vi "GOOP_LVClass_Item_OnPopUpMenu.vi"(11 "Object":u64) -> ()   [LabVIEW 2020]
uses:
  <resource>/Framework/Providers/API/mxLvMenuItem.ctl
  <resource>/Framework/Providers/Open_GDS/ClassProviders/Provider_EndevoGOOP300/EndevoProviderName.ctl
  <resource>/Framework/Providers/Open_GDS/ClassProviders/Provider_EndevoGOOP400/EndevoG4ProviderName.ctl
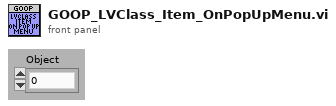
[diagram p1: front panel]
types:
  T1 = typedef "mxLvMenuItem.ctl" = cluster{"Menu Name":string, "Description":string, "Icon File Name":path, "Menu Tag":string, "Enabled":bool, "Checked":bool, "Separator":bool, "Batchable":bool, "Weight":i32, "Batch Mode (Ignored if Not Batchable)":enum32{"Show If All Items Support Command", "Show If Any Items Support Command"}, "Menu Location":enum32{"<None>", "Project", "Project / Build Specifications", "Tools", "Tools / Source Control", "Tools / Real-Time Module", "Help"}, "Exclude From Getting Started Window Menu":bool}
  T2 = typedef "EndevoG4ProviderName.ctl" = enum16{"EndevoGOOP400"}
  T3 = typedef "EndevoProviderName.ctl" = enum16{"EndevoGOOP300"}
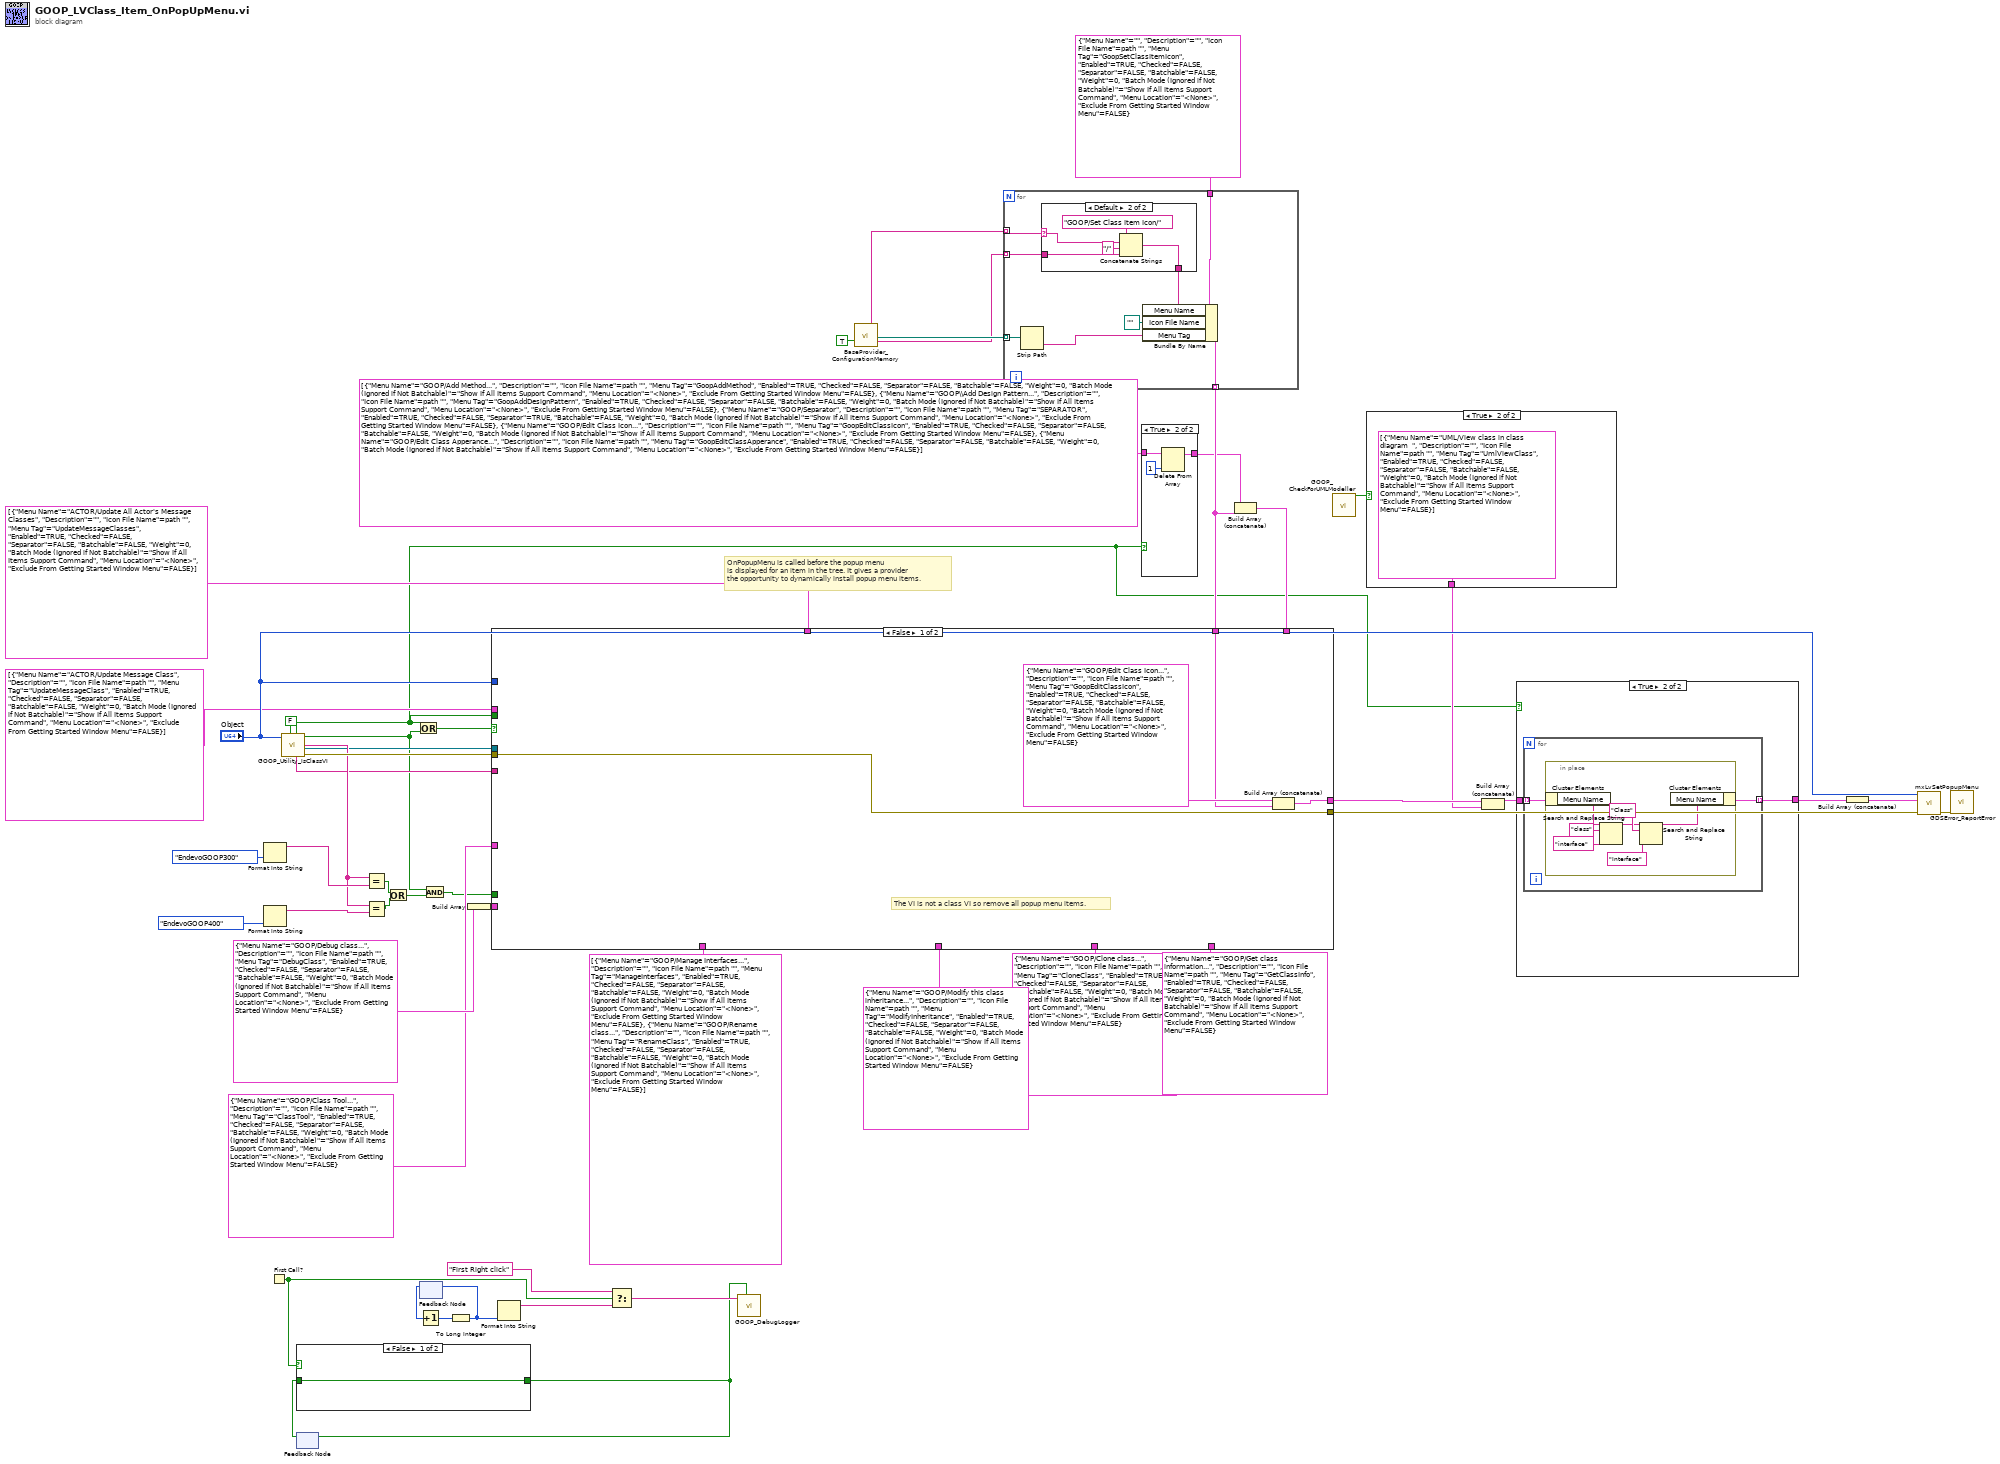
[diagram p0: block diagram]
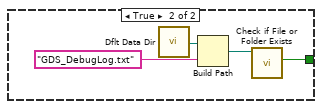
[diagram p5: hidden frame]
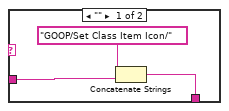
[diagram p6: hidden frame]
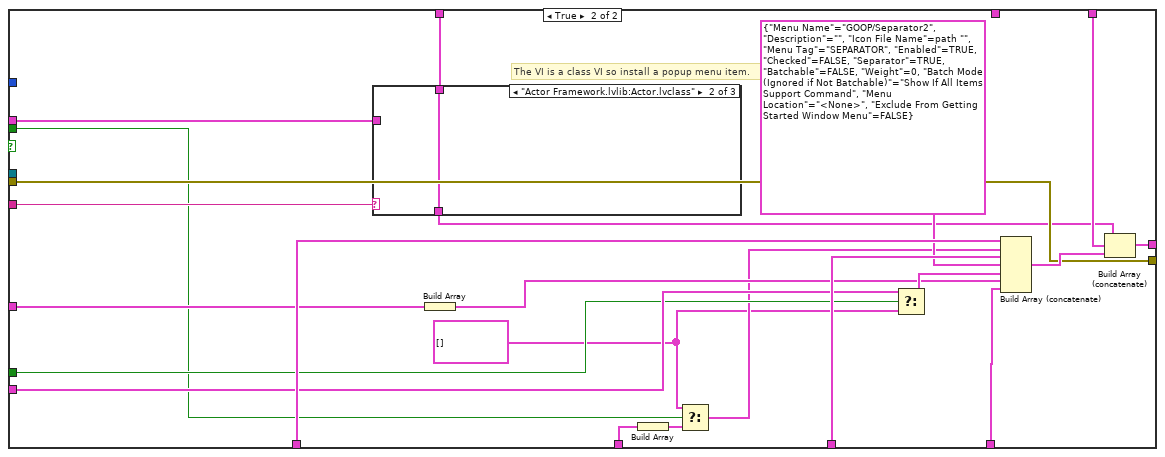
[diagram p7: hidden frame]
diagram:
  # "OnPopupMenu is called before the popup menu\nis displayed for an item in the tree. It gives a provider\nthe opportunity to dynamically install popup menu items."
  n1 = Format Into String(EndevoProviderName."EndevoGOOP300" ("ProviderName")) -> (resulting string=w34:string)  [unwired: 3 in, 1 out]
  n2 = Format Into String(EndevoG4ProviderName."EndevoGOOP400" ("ProviderName")) -> (resulting string=w31:string)  [unwired: 3 in, 1 out]
  n3 = First Call?() -> (First Call?: T/F=w20:bool)
  n4 = call <resource>:"GOOP_Utility_IsClassVI.vi"("KeepClassOpen(False)"=FALSE, "Object"="Object") -> ("error out"=w51:errorcluster, "ClassItem(If Found)"=w13:refnum<vi>, "ClassProvider"=w32:string, "Is Class VI?"=w8:bool, "RootClassQualified Class Name"=w18:string, "Is Interface?"=w3:bool)  [unwired: 4 in]
  n5 = feedback #1() -> (w21:bool)  [unwired: 1 in]
  n6 = case shown="False" w20 {
    tunnel: [w53 w54] -> w19
    tunnel: w21 -> [w53 _]
    frame False {
    }
    frame True {
      n7 = call <vilib>:"Dflt Data Dir.vi"() -> ("App:Default Data Directory"=w56:path)
      n8 = Build Path(base path=w56, name or relative path="GDS_DebugLog.txt") -> (appended path=w57:path)
      n9 = call <vilib>:"Check if File or Folder Exists.vi"("path"=w57) -> ("file or folder exists?"=w54:bool)  [unwired: 8 in, 2 out]
    }
  }
  n10 = feedback-in #1(w19) -> ()
  n11 = Equal?(x=w32, y=w34) -> (x = y?=w29:bool)
  n12 = Equal?(x=w32, y=w31) -> (x = y?=w30:bool)
  n13 = Or(x=w29, y=w30) -> (x .or. y?=w10:bool)
  n14 = Or(x=w3, y=w8) -> (x .or. y?=w11:bool)
  n15 = feedback #2() -> (w25:i32)  [unwired: 1 in]
  n16 = Increment(x=w25) -> (x+1=w24:i32)
  n17 = And(x=w8, y=w10) -> (x .and. y?=w9:bool)
  n18 = To Long Integer(number=w24) -> (32bit integer=w23:i32)
  n19 = feedback-in #2(w23) -> ()
  n20 = Build Array(T1 {"Menu Name"="GOOP/Debug class...", "Description"="", "Icon File Name"=path "", "Menu Tag"="DebugClass", "Enabled"=TRUE, "Checked"=FALSE, "Separator"=FALSE, "Batchable"=FALSE, "Weight"=0, "Batch Mode (Ignored if Not Batchable)"=enum."Show If All Items Support Command", "Menu Location"=enum."<None>", "Exclude From Getting Started Window Menu"=FALSE} ("Menu Item")) -> (w35:T1[])
  n21 = Format Into String(w23) -> (resulting string=w22:string)  [unwired: 3 in, 1 out]
  n22 = Select(t="First Right click" ("name or relative path"), s=w20, f=w22) -> (s? t:f=w27:string)
  n23 = call <resource>:"GOOP_DebugLogger.vi"("ActivateDebugging"=w19, "State"=w27) -> ()  [unwired: 7 in, 3 out]
  n24 = call <resource>:"BaseProvider_ConfigurationMemory.vi"("Filter_Icons"=TRUE) -> ("ClassItemIconGroup"=w28:string[], "ClassItemIconPaths"=w38:path[], "ClassItemIconNames"=w37:string[])  [unwired: 12 in, 4 out]
  n25 = for {
    tunnel: [w64] -> w40 mode=indexing
    tunnel: T1 {"Menu Name"="", "Description"="", "Icon File Name"=path "", "Menu Tag"="GoopSetClassItemIcon", "Enabled"=TRUE, "Checked"=FALSE, "Separator"=FALSE, "Batchable"=FALSE, "Weight"=0, "Batch Mode (Ignored if Not Batchable)"=enum."Show If All Items Support Command", "Menu Location"=enum."<None>", "Exclude From Getting Started Window Menu"=FALSE} ("Menu Item") -> [w65]
    tunnel: w38 -> [w61] mode=indexing
    tunnel: w37 -> [w59] mode=indexing
    tunnel: w28 -> [w58] mode=indexing
    n26 = Strip Path(path=w61) -> (name=w60:string)  [unwired: 1 out]
    n27 = case shown="Default" w58 {
      selector: w58 -> [_ w70]
      tunnel: [w67 w73] -> w62
      tunnel: w59 -> [w66 w72]
      frame "" {
        n28 = Concatenate Strings("GOOP/Set Class Item Icon/" ("string"), w66) -> (w67:string)
      }
      frame Default {
        n29 = Concatenate Strings("GOOP/Set Class Item Icon/" ("string"), w70, "/" ("string"), w72) -> (w73:string)
      }
    }
    n30 = Bundle By Name(cluster=w65, "Menu Name"=w62, "Icon File Name"=path "", "Menu Tag"=w60) -> (w64:T1)
  }
  n31 = case shown="True" w3 {
    tunnel: T1[] [{"Menu Name"="GOOP/Add Method...", "Description"="", "Icon File Name"=path "", "Menu Tag"="GoopAddMethod", "Enabled"=TRUE, "Checked"=FALSE, "Separator"=FALSE, "Batchable"=FALSE, "Weight"=0, "Batch Mode (Ignored if Not Batchable)"=enum."Show If All Items Support Command", "Menu Location"=enum."<None>", "Exclude From Getting Started Window Menu"=FALSE}, {"Menu Name"="GOOP\\Add Design Pattern...", "Description"="", "Icon File Name"=path "", "Menu Tag"="GoopAddDesignPattern", "Enabled"=TRUE, "Checked"=FALSE, "Separator"=FALSE, "Batchable"=FALSE, "Weight"=0, "Batch Mode (Ignored if Not Batchable)"=enum."Show If All Items Support Command", "Menu Location"=enum."<None>", "Exclude From Getting Started Window Menu"=FALSE}, {"Menu Name"="GOOP/Separator", "Description"="", "Icon File Name"=path "", "Menu Tag"="SEPARATOR", "Enabled"=TRUE, "Checked"=FALSE, "Separator"=TRUE, "Batchable"=FALSE, "Weight"=0, "Batch Mode (Ignored if Not Batchable)"=enum."Show If All Items Support Command", "Menu Location"=enum."<None>", "Exclude From Getting Started Window Menu"=FALSE}, {"Menu Name"="GOOP/Edit Class Icon...", "Description"="", "Icon File Name"=path "", "Menu Tag"="GoopEditClassIcon", "Enabled"=TRUE, "Checked"=FALSE, "Separator"=FALSE, "Batchable"=FALSE, "Weight"=0, "Batch Mode (Ignored if Not Batchable)"=enum."Show If All Items Support Command", "Menu Location"=enum."<None>", "Exclude From Getting Started Window Menu"=FALSE}, {"Menu Name"="GOOP/Edit Class Apperance...", "Description"="", "Icon File Name"=path "", "Menu Tag"="GoopEditClassApperance", "Enabled"=TRUE, "Checked"=FALSE, "Separator"=FALSE, "Batchable"=FALSE, "Weight"=0, "Batch Mode (Ignored if Not Batchable)"=enum."Show If All Items Support Command", "Menu Location"=enum."<None>", "Exclude From Getting Started Window Menu"=FALSE}] -> [w74 w77]
    tunnel: [w74 w76] -> w6
    frame False {
    }
    frame True {
      n32 = Delete From Array(array=w77, index=1) -> (array with subset deleted=w76:T1[])  [unwired: 1 in, 1 out]
    }
  }
  n33 = Build Array (concatenate)(w6, w40) -> (w41:T1[])
  n34 = case shown="False" w11 {
    tunnel: [w79 w102] -> w48
    tunnel: "Object" -> [_ _]
    tunnel: w51 -> [w81 w93]
    tunnel: w13 -> [_ _]
    tunnel: T1 {"Menu Name"="GOOP/Modify this class inheritance...", "Description"="", "Icon File Name"=path "", "Menu Tag"="ModifyInheritance", "Enabled"=TRUE, "Checked"=FALSE, "Separator"=FALSE, "Batchable"=FALSE, "Weight"=0, "Batch Mode (Ignored if Not Batchable)"=enum."Show If All Items Support Command", "Menu Location"=enum."<None>", "Exclude From Getting Started Window Menu"=FALSE} ("Menu Item") -> [_ w83]
    tunnel: [w81 w93] -> w14
    tunnel: w41 -> [_ w101]
    tunnel: T1 {"Menu Name"="GOOP/Get class information...", "Description"="", "Icon File Name"=path "", "Menu Tag"="GetClassInfo", "Enabled"=TRUE, "Checked"=FALSE, "Separator"=FALSE, "Batchable"=FALSE, "Weight"=0, "Batch Mode (Ignored if Not Batchable)"=enum."Show If All Items Support Command", "Menu Location"=enum."<None>", "Exclude From Getting Started Window Menu"=FALSE} ("Menu Item") -> [_ w97]
    tunnel: T1[] [{"Menu Name"="GOOP/Manage Interfaces...", "Description"="", "Icon File Name"=path "", "Menu Tag"="ManageInterfaces", "Enabled"=TRUE, "Checked"=FALSE, "Separator"=FALSE, "Batchable"=FALSE, "Weight"=0, "Batch Mode (Ignored if Not Batchable)"=enum."Show If All Items Support Command", "Menu Location"=enum."<None>", "Exclude From Getting Started Window Menu"=FALSE}, {"Menu Name"="GOOP/Rename class...", "Description"="", "Icon File Name"=path "", "Menu Tag"="RenameClass", "Enabled"=TRUE, "Checked"=FALSE, "Separator"=FALSE, "Batchable"=FALSE, "Weight"=0, "Batch Mode (Ignored if Not Batchable)"=enum."Show If All Items Support Command", "Menu Location"=enum."<None>", "Exclude From Getting Started Window Menu"=FALSE}] ("Array") -> [_ w100]
    tunnel: T1 {"Menu Name"="GOOP/Clone class...", "Description"="", "Icon File Name"=path "", "Menu Tag"="CloneClass", "Enabled"=TRUE, "Checked"=FALSE, "Separator"=FALSE, "Batchable"=FALSE, "Weight"=0, "Batch Mode (Ignored if Not Batchable)"=enum."Show If All Items Support Command", "Menu Location"=enum."<None>", "Exclude From Getting Started Window Menu"=FALSE} ("Menu Item") -> [_ w99]
    tunnel: w35 -> [_ w95]
    tunnel: w40 -> [w78 _]
    tunnel: w9 -> [_ w94]
    tunnel: w18 -> [_ w92]
    tunnel: T1[] [{"Menu Name"="ACTOR/Update All Actor's Message Classes", "Description"="", "Icon File Name"=path "", "Menu Tag"="UpdateMessageClasses", "Enabled"=TRUE, "Checked"=FALSE, "Separator"=FALSE, "Batchable"=FALSE, "Weight"=0, "Batch Mode (Ignored if Not Batchable)"=enum."Show If All Items Support Command", "Menu Location"=enum."<None>", "Exclude From Getting Started Window Menu"=FALSE}] -> [_ w91]
    tunnel: T1[] [{"Menu Name"="ACTOR/Update Message Class", "Description"="", "Icon File Name"=path "", "Menu Tag"="UpdateMessageClass", "Enabled"=TRUE, "Checked"=FALSE, "Separator"=FALSE, "Batchable"=FALSE, "Weight"=0, "Batch Mode (Ignored if Not Batchable)"=enum."Show If All Items Support Command", "Menu Location"=enum."<None>", "Exclude From Getting Started Window Menu"=FALSE}] -> [_ w90]
    tunnel: T1 {"Menu Name"="GOOP/Class Tool...", "Description"="", "Icon File Name"=path "", "Menu Tag"="ClassTool", "Enabled"=TRUE, "Checked"=FALSE, "Separator"=FALSE, "Batchable"=FALSE, "Weight"=0, "Batch Mode (Ignored if Not Batchable)"=enum."Show If All Items Support Command", "Menu Location"=enum."<None>", "Exclude From Getting Started Window Menu"=FALSE} ("Menu Item") -> [_ w87]
    tunnel: w3 -> [_ w86]
    frame False {
      # "The VI is not a class VI so remove all popup menu items."
      n35 = Build Array (concatenate)(T1 {"Menu Name"="GOOP/Edit Class Icon...", "Description"="", "Icon File Name"=path "", "Menu Tag"="GoopEditClassIcon", "Enabled"=TRUE, "Checked"=FALSE, "Separator"=FALSE, "Batchable"=FALSE, "Weight"=0, "Batch Mode (Ignored if Not Batchable)"=enum."Show If All Items Support Command", "Menu Location"=enum."<None>", "Exclude From Getting Started Window Menu"=FALSE} ("Menu Item"), w78) -> (w79:T1[])
    }
    frame True {
      w82 = T1[] []
      # "The VI is a class VI so install a popup menu item."
      n36 = case shown="\"Actor Framework.lvlib:Actor.lvclass\"" w92 {
        tunnel: w91 -> [_ w104 _]
        tunnel: [_ w104 w105] -> w89
        tunnel: w90 -> [_ _ w105]
        frame Default {
        }
        frame "Actor Framework.lvlib:Actor.lvclass" {
        }
        frame "Actor Framework.lvlib:Message.lvclass" {
        }
      }
      n37 = Build Array(w87) -> (w88:T1[])
      n38 = Build Array(w83) -> (w85:T1[])
      n39 = Select(t=w82, s=w86, f=w85) -> (s? t:f=w84:T1[])
      n40 = Select(t=w95, s=w94, f=w82) -> (s? t:f=w96:T1[])
      n41 = Build Array (concatenate)(w100, w84, w99, T1 {"Menu Name"="GOOP/Separator2", "Description"="", "Icon File Name"=path "", "Menu Tag"="SEPARATOR", "Enabled"=TRUE, "Checked"=FALSE, "Separator"=TRUE, "Batchable"=FALSE, "Weight"=0, "Batch Mode (Ignored if Not Batchable)"=enum."Show If All Items Support Command", "Menu Location"=enum."<None>", "Exclude From Getting Started Window Menu"=FALSE} ("Menu Item"), w96, w88, w97) -> (w103:T1[])
      n42 = Build Array (concatenate)(w89, w101, w103) -> (w102:T1[])
    }
  }
  n43 = call <resource>:"GOOP_CheckForUMLModeller.vi"() -> ("UML Modeller Exists"=w2:bool)  [unwired: 10 in, 1 out]
  n44 = case shown="True" w2 {
    tunnel: [_ T1[] [{"Menu Name"="UML/View class in class diagram  ", "Description"="", "Icon File Name"=path "", "Menu Tag"="UmlViewClass", "Enabled"=TRUE, "Checked"=FALSE, "Separator"=FALSE, "Batchable"=FALSE, "Weight"=0, "Batch Mode (Ignored if Not Batchable)"=enum."Show If All Items Support Command", "Menu Location"=enum."<None>", "Exclude From Getting Started Window Menu"=FALSE}]] -> w47
    frame False {
    }
    frame True {
    }
  }
  n45 = Build Array (concatenate)(w48, w47) -> (w5:T1[])
  n46 = case shown="True" w3 {
    tunnel: w5 -> [w107 w109]
    tunnel: [w107 w108] -> w4
    frame False {
    }
    frame True {
      n47 = for {
        tunnel: w109 -> [w111] mode=indexing
        tunnel: [w110] -> w108 mode=indexing
        n48 = in-place {
          n49 = in-place-cluster #3(w111) -> ("Menu Name"=w118:string)
          n50 = Search and Replace String(input string=w118, search string="class", replace string="interface" ("replace string (\"\")")) -> (result string=w113:string)  [unwired: 5 in, 3 out]
          n51 = Search and Replace String(input string=w113, search string="Class", replace string="Interface" ("replace string (\"\")")) -> (result string=w112:string)  [unwired: 5 in, 3 out]
          n52 = in-place-cluster #3("Menu Name"=w112) -> (w110:T1)
        }
      }
    }
  }
  n53 = Build Array (concatenate)(w4) -> (w1:T1[])
  n54 = call <resource>:"mxLvSetPopupMenu.vi"("error in"=w14, "Popup Menu Items"=w1, "Item"="Object") -> ("error out"=w44:errorcluster)  [unwired: 7 in, 1 out]
  n55 = call <resource>:"GDSError_ReportError.vi"("error in (no error)"=w44) -> ()  [unwired: 18 in, 1 out]
